vi "IsSeparator.vi"(8 "error in (no error)":errorcluster, 11 "Separator in":refnum<class "Separator.lvclass">) -> (0 "error out":errorcluster, 2 "separator?":bool, 3 "Separator out":refnum<class "Separator.lvclass">)   [LabVIEW 2023, in "GettingStartedWindow.lvlib" / "Separator.lvclass"]
uses:
  <resource>/modes/FRC/Classes/Separator/Separator.lvclass
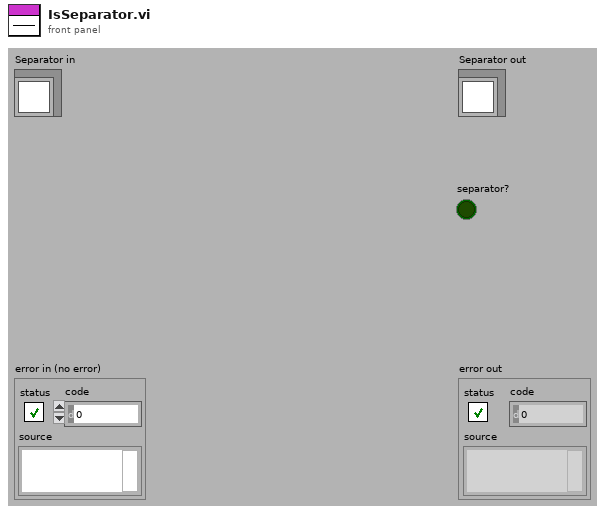
[diagram p1: front panel]
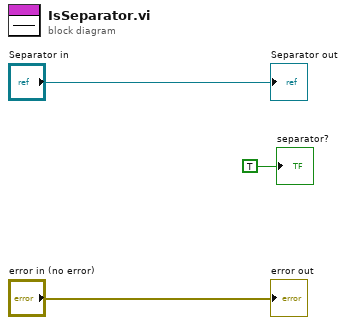
[diagram p0: block diagram]
diagram:
  "error out" <- "error in (no error)"
  "Separator out" <- "Separator in"
  "separator?" <- TRUE ("separator?")
